vi "Test Read-Write Control Text.vi"(8 "error in (no error)":errorcluster) -> (0 "error out":errorcluster, 3 "Pass?":bool)   [LabVIEW 2020]
uses:
  G-Unicode/Unicode/Controls/String Encoding.ctl
  G-Unicode/Types/UTF-8 String/UTF-8 String.lvclass/UTF-8 String.ctl
  5655a432-7152-4618-8a1b-1a6feeb00f3f.vi
  G-Unicode/Dialog & User Interface/Polymorphic VIs/Write Control Text/Write Listbox Header (UTF-8 String).vi
  G-Unicode/Dialog & User Interface/Polymorphic VIs/Read Control Text/Read Listbox Header (UTF-8 String).vi
  47e1521e-4900-4e50-93d0-971907de44b7.vi
  G-Unicode/Dialog & User Interface/Polymorphic VIs/Write Control Text/Write Graph Plot Names (UTF-8 String).vi
  G-Unicode/Dialog & User Interface/Polymorphic VIs/Write Control Text/Write Graph Cursor Names (UTF-8 String).vi
  G-Unicode/Dialog & User Interface/Polymorphic VIs/Write Control Text/Write Graph Axis Labels (UTF-8 String).vi
  G-Unicode/Dialog & User Interface/Polymorphic VIs/Write Control Text/Write Table Headers (UTF-8 String).vi
  G-Unicode/Dialog & User Interface/Polymorphic VIs/Read Control Text/Read Table Headers (UTF-8 String).vi
  cbd299b7-ed5c-44d8-98e3-4b07b256a3af.vi
  97e6e9dd-fb41-465e-8130-768105b8566a.vi
  G-Unicode/Dialog & User Interface/Polymorphic VIs/Write Control Text/Write Multicolumn Listbox Headers (UTF-8 String).vi
  G-Unicode/Dialog & User Interface/Polymorphic VIs/Read Control Text/Read Multicolumn Listbox Headers (UTF-8 String).vi
  2cb1db3a-9545-49da-8e46-b28431192bfb.vi
  d3ca7cbe-fe55-4c08-9226-8df1279bea32.vi
  G-Unicode/Dialog & User Interface/Polymorphic VIs/Write Control Text/Write Radio Button Text (UTF-8 String).vi
  G-Unicode/Dialog & User Interface/Polymorphic VIs/Read Control Text/Read Radio Button Text (UTF-8 String).vi
  c66c8a8e-6384-46dd-ad34-c6b36e981c5f.vi
  G-Unicode/Dialog & User Interface/Polymorphic VIs/Write Control Text/Write Tab Pages (UTF-8 String).vi
  G-Unicode/Dialog & User Interface/Polymorphic VIs/Read Control Text/Read Tab Pages (UTF-8 String).vi
  11ce0e2c-e1a8-46a3-af78-7df26efc8245.vi
  G-Unicode/Dialog & User Interface/Polymorphic VIs/Write Control Text/Write Listbox Items (UTF-8 String).vi
  G-Unicode/Dialog & User Interface/Polymorphic VIs/Read Control Text/Read Listbox Items (UTF-8 String).vi
  c5b5f753-7993-4590-ab7a-38cd070e680f.vi
  G-Unicode/Dialog & User Interface/Polymorphic VIs/Write Control Text/Write Table Value (UTF-8 String).vi
  G-Unicode/Dialog & User Interface/Polymorphic VIs/Read Control Text/Read Table Value (UTF-8 String).vi
  d87d6912-68ee-4c4f-8e1f-9eaf2c3e8737.vi
  G-Unicode/Dialog & User Interface/Polymorphic VIs/Write Control Text/Write Ring Strings (UTF-8 String).vi
  G-Unicode/Dialog & User Interface/Polymorphic VIs/Read Control Text/Read Ring Strings (UTF-8 String).vi
  b51df372-b908-46a9-9cd9-1bce9bcba761.vi
  3f50c59c-438d-4159-8265-e7e5e4819d1d.vi
  G-Unicode/Dialog & User Interface/Polymorphic VIs/Write Control Text/Write 2D String Array Value (UTF-8 String).vi
  G-Unicode/Dialog & User Interface/Polymorphic VIs/Read Control Text/Read 2D String Array Value (UTF-8 String).vi
  f481c7ac-37a4-4879-9d59-93dd94c77838.vi
  G-Unicode/Dialog & User Interface/Polymorphic VIs/Write Control Text/Write 1D String Array Value (UTF-8 String).vi
  G-Unicode/Dialog & User Interface/Polymorphic VIs/Read Control Text/Read 1D String Array Value (UTF-8 String).vi
  2abff34c-ba54-40bb-bfb0-e7a9eb1a66c8.vi
  G-Unicode/Dialog & User Interface/Polymorphic VIs/Write Control Text/Write String Value (UTF-8 String).vi
  G-Unicode/Dialog & User Interface/Polymorphic VIs/Read Control Text/Read String Value (UTF-8 String).vi
  b9bba32d-5ca2-4258-b841-0da24b58b874.vi
  G-Unicode/Dialog & User Interface/Polymorphic VIs/Write Control Text/Write Multicolumn Listbox Items (UTF-8 String).vi
  G-Unicode/Dialog & User Interface/Polymorphic VIs/Read Control Text/Read Multicolumn Listbox Items (UTF-8 String).vi
  4c20338b-6e60-4a75-91ad-9e96f58f92b0.vi
  G-Unicode/Unicode/Encode String.vi
  5655a432-7152-4618-8a1b-1a6feeb00f3f.vi/46bf550a-28c6-4dfd-813a-9b0ad34779ef.vi
  G-Unicode/Private/Conversion/String as Encoded String.vi
  G-Unicode/Private/Conversion/Polymorphic VIs/String as Encoded String (UTF-8 String).vi
  G-Unicode/Types/UTF-8 String/Write Encoded UTF-8 String.vi
  G-Unicode/Dialog & User Interface/Polymorphic VIs/Write Control Text/Write Listbox Header (UTF-8 String).vi/5206cb6b-04fb-41f5-a37e-29c14f142303.vi
  G-Unicode/Dialog & User Interface/Polymorphic VIs/Read Control Text/Read Listbox Header (UTF-8 String).vi/bfba3187-b22e-4285-8cc2-1816a803f974.vi
  47e1521e-4900-4e50-93d0-971907de44b7.vi/3a31b270-3bb6-4c58-a256-c5fcc2c98f09.vi
  47e1521e-4900-4e50-93d0-971907de44b7.vi/0ec5df2d-ef9b-4f84-a6a8-ffcedd45c4dc.vi
  G-Unicode/Dialog & User Interface/Polymorphic VIs/Write Control Text/Write Graph Plot Names (UTF-8 String).vi/5206cb6b-04fb-41f5-a37e-29c14f142303.vi
  G-Unicode/Dialog & User Interface/Polymorphic VIs/Write Control Text/Write Graph Cursor Names (UTF-8 String).vi/5206cb6b-04fb-41f5-a37e-29c14f142303.vi
  G-Unicode/Dialog & User Interface/Polymorphic VIs/Write Control Text/Write Graph Axis Labels (UTF-8 String).vi/5206cb6b-04fb-41f5-a37e-29c14f142303.vi
  G-Unicode/Dialog & User Interface/Polymorphic VIs/Write Control Text/Write Graph Axis Labels (UTF-8 String).vi/dd8e371b-806c-4d03-8f90-d02a4c0388fb.vi
  G-Unicode/Dialog & User Interface/Polymorphic VIs/Write Control Text/Write Table Headers (UTF-8 String).vi/5206cb6b-04fb-41f5-a37e-29c14f142303.vi
  G-Unicode/Dialog & User Interface/Polymorphic VIs/Write Control Text/Write Table Headers (UTF-8 String).vi/ac01c1c3-6448-4046-bb74-48d1977bc508.vi
  G-Unicode/Dialog & User Interface/Polymorphic VIs/Read Control Text/Read Table Headers (UTF-8 String).vi/f6f7f231-7ddf-476b-a943-0386d848a5c9.vi
  G-Unicode/Dialog & User Interface/Polymorphic VIs/Read Control Text/Read Table Headers (UTF-8 String).vi/fba5a6d2-cdfe-4afc-9e2c-d2641906be0d.vi
  cbd299b7-ed5c-44d8-98e3-4b07b256a3af.vi/3a31b270-3bb6-4c58-a256-c5fcc2c98f09.vi
  cbd299b7-ed5c-44d8-98e3-4b07b256a3af.vi/0ec5df2d-ef9b-4f84-a6a8-ffcedd45c4dc.vi
  97e6e9dd-fb41-465e-8130-768105b8566a.vi/3a31b270-3bb6-4c58-a256-c5fcc2c98f09.vi
  97e6e9dd-fb41-465e-8130-768105b8566a.vi/0ec5df2d-ef9b-4f84-a6a8-ffcedd45c4dc.vi
  G-Unicode/Dialog & User Interface/Polymorphic VIs/Write Control Text/Write Multicolumn Listbox Headers (UTF-8 String).vi/5206cb6b-04fb-41f5-a37e-29c14f142303.vi
  G-Unicode/Dialog & User Interface/Polymorphic VIs/Write Control Text/Write Multicolumn Listbox Headers (UTF-8 String).vi/ac01c1c3-6448-4046-bb74-48d1977bc508.vi
  G-Unicode/Dialog & User Interface/Polymorphic VIs/Read Control Text/Read Multicolumn Listbox Headers (UTF-8 String).vi/f6f7f231-7ddf-476b-a943-0386d848a5c9.vi
  G-Unicode/Dialog & User Interface/Polymorphic VIs/Read Control Text/Read Multicolumn Listbox Headers (UTF-8 String).vi/fba5a6d2-cdfe-4afc-9e2c-d2641906be0d.vi
  2cb1db3a-9545-49da-8e46-b28431192bfb.vi/3a31b270-3bb6-4c58-a256-c5fcc2c98f09.vi
  2cb1db3a-9545-49da-8e46-b28431192bfb.vi/0ec5df2d-ef9b-4f84-a6a8-ffcedd45c4dc.vi
  d3ca7cbe-fe55-4c08-9226-8df1279bea32.vi/3a31b270-3bb6-4c58-a256-c5fcc2c98f09.vi
  d3ca7cbe-fe55-4c08-9226-8df1279bea32.vi/0ec5df2d-ef9b-4f84-a6a8-ffcedd45c4dc.vi
  G-Unicode/Dialog & User Interface/Polymorphic VIs/Write Control Text/Write Radio Button Text (UTF-8 String).vi/5206cb6b-04fb-41f5-a37e-29c14f142303.vi
  G-Unicode/Dialog & User Interface/Polymorphic VIs/Read Control Text/Read Radio Button Text (UTF-8 String).vi/f6f7f231-7ddf-476b-a943-0386d848a5c9.vi
  c66c8a8e-6384-46dd-ad34-c6b36e981c5f.vi/3a31b270-3bb6-4c58-a256-c5fcc2c98f09.vi
  c66c8a8e-6384-46dd-ad34-c6b36e981c5f.vi/0ec5df2d-ef9b-4f84-a6a8-ffcedd45c4dc.vi
  G-Unicode/Dialog & User Interface/Polymorphic VIs/Write Control Text/Write Tab Pages (UTF-8 String).vi/5206cb6b-04fb-41f5-a37e-29c14f142303.vi
  G-Unicode/Dialog & User Interface/Polymorphic VIs/Read Control Text/Read Tab Pages (UTF-8 String).vi/f6f7f231-7ddf-476b-a943-0386d848a5c9.vi
  11ce0e2c-e1a8-46a3-af78-7df26efc8245.vi/3a31b270-3bb6-4c58-a256-c5fcc2c98f09.vi
  11ce0e2c-e1a8-46a3-af78-7df26efc8245.vi/0ec5df2d-ef9b-4f84-a6a8-ffcedd45c4dc.vi
  G-Unicode/Dialog & User Interface/Polymorphic VIs/Write Control Text/Write Listbox Items (UTF-8 String).vi/5206cb6b-04fb-41f5-a37e-29c14f142303.vi
  G-Unicode/Dialog & User Interface/Polymorphic VIs/Read Control Text/Read Listbox Items (UTF-8 String).vi/f6f7f231-7ddf-476b-a943-0386d848a5c9.vi
  c5b5f753-7993-4590-ab7a-38cd070e680f.vi/3a31b270-3bb6-4c58-a256-c5fcc2c98f09.vi
  c5b5f753-7993-4590-ab7a-38cd070e680f.vi/0ec5df2d-ef9b-4f84-a6a8-ffcedd45c4dc.vi
  G-Unicode/Dialog & User Interface/Polymorphic VIs/Write Control Text/Write Table Value (UTF-8 String).vi/5206cb6b-04fb-41f5-a37e-29c14f142303.vi
  G-Unicode/Dialog & User Interface/Polymorphic VIs/Read Control Text/Read Table Value (UTF-8 String).vi/f6f7f231-7ddf-476b-a943-0386d848a5c9.vi
  d87d6912-68ee-4c4f-8e1f-9eaf2c3e8737.vi/3a31b270-3bb6-4c58-a256-c5fcc2c98f09.vi
  d87d6912-68ee-4c4f-8e1f-9eaf2c3e8737.vi/0ec5df2d-ef9b-4f84-a6a8-ffcedd45c4dc.vi
  G-Unicode/Dialog & User Interface/Polymorphic VIs/Write Control Text/Write Ring Strings (UTF-8 String).vi/5206cb6b-04fb-41f5-a37e-29c14f142303.vi
  G-Unicode/Dialog & User Interface/Polymorphic VIs/Read Control Text/Read Ring Strings (UTF-8 String).vi/f6f7f231-7ddf-476b-a943-0386d848a5c9.vi
  b51df372-b908-46a9-9cd9-1bce9bcba761.vi/3a31b270-3bb6-4c58-a256-c5fcc2c98f09.vi
  b51df372-b908-46a9-9cd9-1bce9bcba761.vi/0ec5df2d-ef9b-4f84-a6a8-ffcedd45c4dc.vi
  3f50c59c-438d-4159-8265-e7e5e4819d1d.vi/3a31b270-3bb6-4c58-a256-c5fcc2c98f09.vi
  3f50c59c-438d-4159-8265-e7e5e4819d1d.vi/0ec5df2d-ef9b-4f84-a6a8-ffcedd45c4dc.vi
  G-Unicode/Dialog & User Interface/Polymorphic VIs/Write Control Text/Write 2D String Array Value (UTF-8 String).vi/5206cb6b-04fb-41f5-a37e-29c14f142303.vi
  G-Unicode/Dialog & User Interface/Polymorphic VIs/Read Control Text/Read 2D String Array Value (UTF-8 String).vi/f6f7f231-7ddf-476b-a943-0386d848a5c9.vi
  f481c7ac-37a4-4879-9d59-93dd94c77838.vi/3a31b270-3bb6-4c58-a256-c5fcc2c98f09.vi
  f481c7ac-37a4-4879-9d59-93dd94c77838.vi/0ec5df2d-ef9b-4f84-a6a8-ffcedd45c4dc.vi
  G-Unicode/Dialog & User Interface/Polymorphic VIs/Write Control Text/Write 1D String Array Value (UTF-8 String).vi/5206cb6b-04fb-41f5-a37e-29c14f142303.vi
  G-Unicode/Dialog & User Interface/Polymorphic VIs/Read Control Text/Read 1D String Array Value (UTF-8 String).vi/f6f7f231-7ddf-476b-a943-0386d848a5c9.vi
  2abff34c-ba54-40bb-bfb0-e7a9eb1a66c8.vi/3a31b270-3bb6-4c58-a256-c5fcc2c98f09.vi
  2abff34c-ba54-40bb-bfb0-e7a9eb1a66c8.vi/0ec5df2d-ef9b-4f84-a6a8-ffcedd45c4dc.vi
  G-Unicode/Dialog & User Interface/Polymorphic VIs/Write Control Text/Write String Value (UTF-8 String).vi/5206cb6b-04fb-41f5-a37e-29c14f142303.vi
  G-Unicode/Dialog & User Interface/Polymorphic VIs/Read Control Text/Read String Value (UTF-8 String).vi/bfba3187-b22e-4285-8cc2-1816a803f974.vi
  b9bba32d-5ca2-4258-b841-0da24b58b874.vi/3a31b270-3bb6-4c58-a256-c5fcc2c98f09.vi
  b9bba32d-5ca2-4258-b841-0da24b58b874.vi/0ec5df2d-ef9b-4f84-a6a8-ffcedd45c4dc.vi
  G-Unicode/Dialog & User Interface/Polymorphic VIs/Write Control Text/Write Multicolumn Listbox Items (UTF-8 String).vi/5206cb6b-04fb-41f5-a37e-29c14f142303.vi
  G-Unicode/Dialog & User Interface/Polymorphic VIs/Read Control Text/Read Multicolumn Listbox Items (UTF-8 String).vi/f6f7f231-7ddf-476b-a943-0386d848a5c9.vi
  4c20338b-6e60-4a75-91ad-9e96f58f92b0.vi/3a31b270-3bb6-4c58-a256-c5fcc2c98f09.vi
  4c20338b-6e60-4a75-91ad-9e96f58f92b0.vi/0ec5df2d-ef9b-4f84-a6a8-ffcedd45c4dc.vi
  G-Unicode/Private/Conversion/Text to UTF-8.vi
  G-Unicode/Private/Conversion/Polymorphic VIs/Text to UTF-8 (LabVIEW String).vi
  G-Unicode/Private/Conversion/Encoded UTF-8 String to Encoded UTF-16LE String.vi
  G-Unicode/Unicode/SubVIs/UTF-16 Byte Swap.vi
  G-Unicode/Private/Conversion/UTF-8 to Text.vi
  G-Unicode/Private/Conversion/Polymorphic VIs/UTF-8 to Text (LabVIEW String).vi
  G-Unicode/Private/Conversion/Encoded UTF-16LE String to Encoded UTF-8 String.vi
  G-Unicode/Unicode/Prepend BOM.vi
  G-Unicode/Private/Conversion/Polymorphic VIs/String as Encoded String (LabVIEW String).vi
  G-Unicode/Types/UTF-8 String/Read Encoded UTF-8 String.vi
  G-Unicode/Private/Conversion/Text as Encoded String.vi
  G-Unicode/Private/Conversion/Polymorphic VIs/Text as Encoded String (UTF-8 String).vi
  G-Unicode/Unicode/SubVIs/Byte Order Marks.vi
  G-Unicode/Unicode/Detect BOM.vi
  G-Unicode/Unicode/Detect String Encoding.vi
  G-Unicode/Private/User Interface/Write String.vi
  G-Unicode/Private/User Interface/Read String.vi
  G-Unicode/Private/User Interface/Write String Array (1D).vi
  G-Unicode/Private/User Interface/Read String Array (1D).vi
  G-Unicode/Private/User Interface/Write String Array (2D).vi
  G-Unicode/Private/User Interface/Read String Array (2D).vi
  G-Unicode/Private/User Interface/Write Ring Control.vi
  G-Unicode/Private/User Interface/Read Ring Control.vi
  G-Unicode/Private/User Interface/Write MultCol Listbox Data.vi
  G-Unicode/Private/User Interface/Read MultCol Listbox Data.vi
  G-Unicode/Private/User Interface/Write MultCol Listbox Headers.vi
  G-Unicode/Private/User Interface/Read MultCol Listbox Headers.vi
  G-Unicode/Private/User Interface/Write Listbox Data.vi
  G-Unicode/Private/User Interface/Read Listbox Data.vi
  G-Unicode/Private/User Interface/Write Listbox Header.vi
  G-Unicode/Private/User Interface/Read Listbox Header.vi
  G-Unicode/Private/User Interface/Write Table Data.vi
  G-Unicode/Private/User Interface/Read Table Data.vi
  G-Unicode/Private/User Interface/Write Table Headers.vi
  G-Unicode/Private/User Interface/Read Table Headers.vi
  G-Unicode/Private/User Interface/Write Tab Control.vi
  G-Unicode/Private/User Interface/Read Tab Control.vi
  G-Unicode/Private/User Interface/Write Radio Buttons.vi
  G-Unicode/Private/User Interface/Read Radio Button Text.vi
  G-Unicode/Private/User Interface/Write Graph-Chart Plot Names.vi
  G-Unicode/Private/User Interface/Write Graph-Chart Axis Labels.vi
  G-Unicode/Private/User Interface/Write Graph-Chart Cursor Names.vi
  G-Unicode/Types/UTF-8 String/UTF-8 String.lvclass
  G-Unicode/G-Unicode.lvlib
panel:
  out "Waveform Graph":dbl[](graph)
  out "Waveform Chart":dbl(graph)
  in  "Radio Buttons":T1(radio)
  in  "Tab Control":enum32{"Page 1", "Page 2", "Page 3", "Page 4"}(tab)
  in  "Multicolumn Listbox":i32(listbox)
  in  "Listbox":i32(listbox)
  in  "Table Control":string[][](table)
  in  "Menu Ring":u16(ring)
  in  "Text Ring":u16(ring)
  in  "String Array (2D)":string[][](array[string])
  in  "String Array (1D)":string[](array[string])
  in  "String":string
  # "Note the dropdowns for the ring controls aren't rendered correctly, but when selected it looks OK."
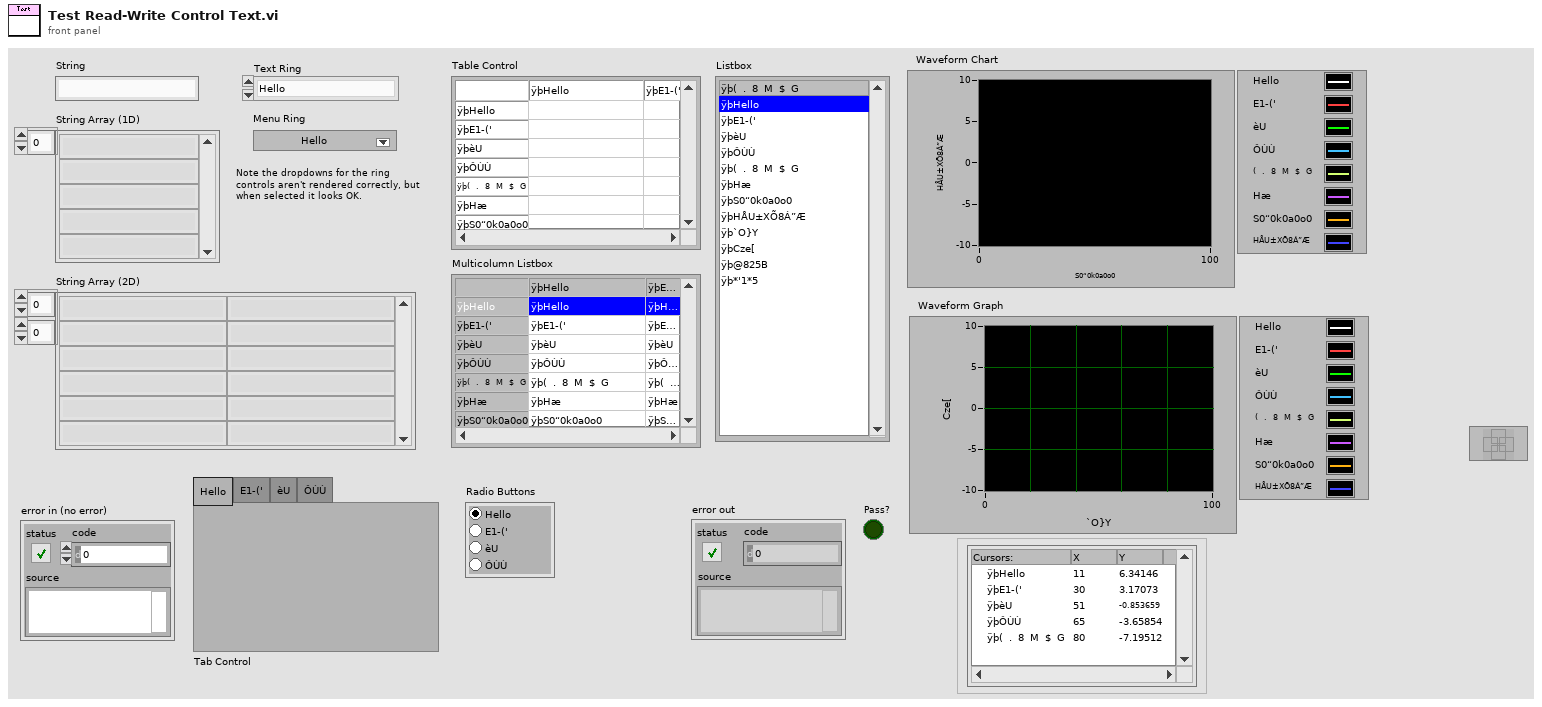
[diagram p1: front panel]
types:
  T1 = enum32{"Radio Selection 1", "Radio Selection 2", "Radio Selection 3", "Radio Selection 4"}
  T2 = typedef "G-Unicode.lvlib/String Encoding.ctl" = enum16{"ANSI", "UTF-8", "UTF-16LE", "UTF-16BE", "Unknown"}
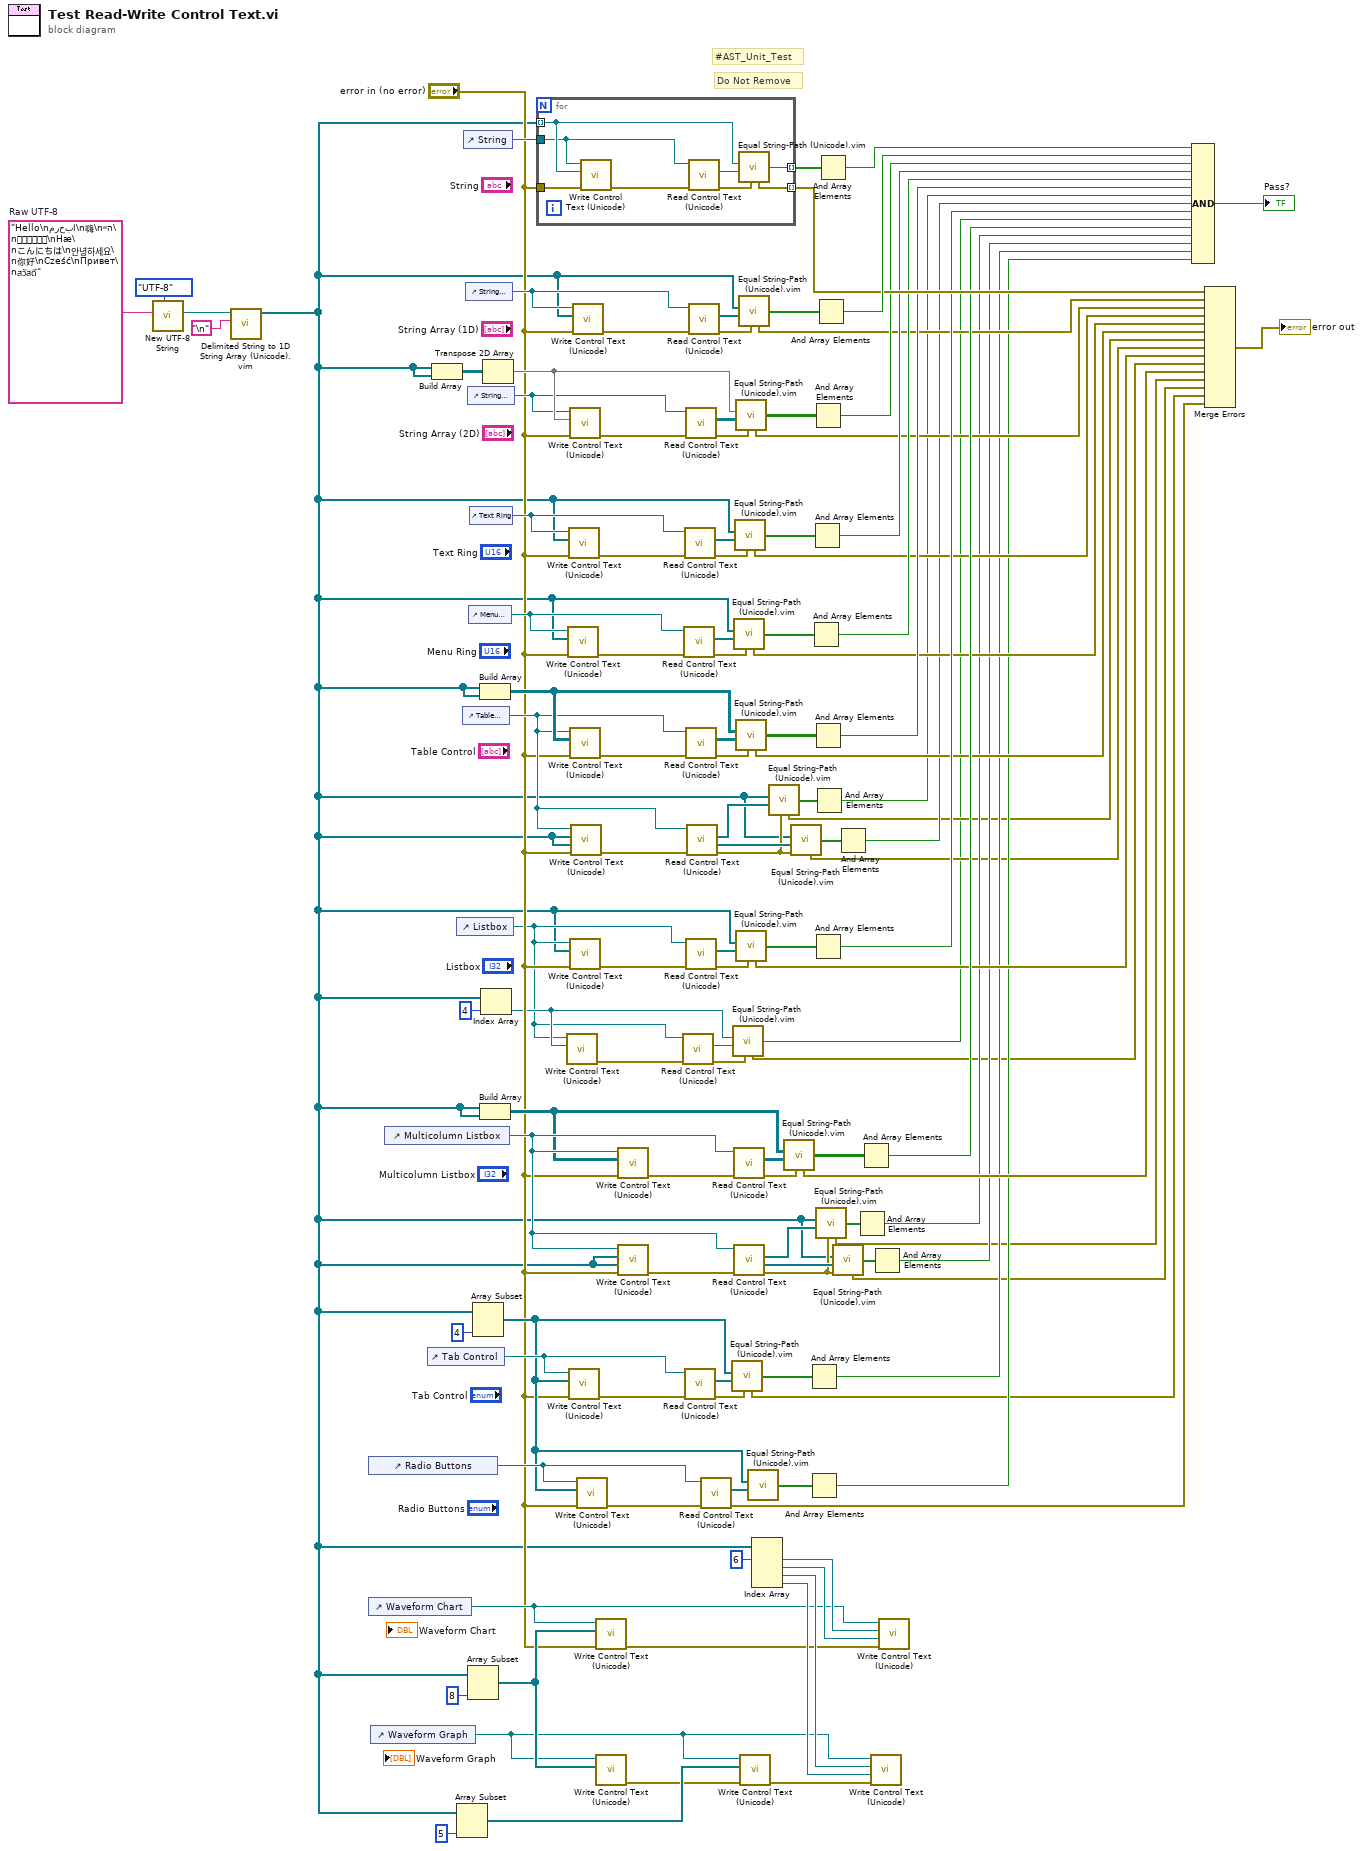
[diagram p0: block diagram]
diagram:
  w2 = "Hello\nمرحبا\n嗨\nהיי\nनमस्ते\nHæ\nこんにちは\n안녕하세요\n你好\nCześć\nПривет\nสวัสดี"  # Raw UTF-8
  # "Do Not Remove"
  # "#AST_Unit_Test"
  n1 = call "New UTF-8 String.vi"("Input Encoding (ANSI)"=String_Encoding."UTF-8", "String"=w2) -> ("UTF-8 String"=w4:refnum<class "UTF-8 String.lvclass">)  [unwired: 8 in, 1 out]
  n2 = call "Delimited String to 1D String Array (Unicode).vim"("Delimiter (tab)"="\n", "Delimited String"=w4) -> ("String Array"=w1:refnum<class "UTF-8 String.lvclass">[])  [unwired: 8 in, 1 out]
  n3 = control-ref of="Radio Buttons"() -> (w44:refnum<vi>)
  n4 = control-ref of="Waveform Chart"() -> (w52:refnum<vi>)
  n5 = control-ref of="Waveform Graph"() -> (w56:refnum<vi>)
  n6 = control-ref of="Multicolumn Listbox"() -> (w41:refnum<vi>)
  n7 = control-ref of="Tab Control"() -> (w47:refnum<vi>)
  n8 = Build Array(w1, w1) -> (w108:refnum<class "UTF-8 String.lvclass">[][])
  n9 = control-ref of="Listbox"() -> (w8:refnum<vi>)
  n10 = Array Subset(array=w1, length=5) -> (w64:refnum<class "UTF-8 String.lvclass">[])  [unwired: 1 in]
  n11 = control-ref of="Table Control"() -> (w26:refnum<vi>)
  n12 = control-ref of="String"() -> (w121:refnum<vi>)
  n13 = control-ref of="String Array (1D)"() -> (w51:refnum<vi>)
  n14 = control-ref of="String Array (2D)"() -> (w50:refnum<vi>)
  n15 = Array Subset(array=w1, length=8) -> (w62:refnum<class "UTF-8 String.lvclass">[])  [unwired: 1 in]
  n16 = control-ref of="Menu Ring"() -> (w48:refnum<vi>)
  n17 = control-ref of="Text Ring"() -> (w49:refnum<vi>)
  n18 = Array Subset(array=w1, length=4) -> (w43:refnum<class "UTF-8 String.lvclass">[])  [unwired: 1 in]
  n19 = Build Array(w1, w1) -> (w94:refnum<class "UTF-8 String.lvclass">[][])
  n20 = Build Array(w1, w1) -> (w40:refnum<class "UTF-8 String.lvclass">[][])
  n21 = Index Array(array=w1, index=4) -> (element=w9:refnum<class "UTF-8 String.lvclass">)
  n22 = Transpose 2D Array(2D array=w108) -> (transposed array=w106:refnum<class "UTF-8 String.lvclass">[][])
  n23 = for {
    tunnel: w121 -> [w122]
    tunnel: w1 -> [w124] mode=indexing
    tunnel: "error in (no error)" -> [w128]
    tunnel: [w125] -> w112 mode=indexing
    tunnel: [w127] -> w120 mode=indexing
    n24 = call-poly "Write Control Text (Unicode).vi"("error in"=w128, "Value"=w124, "Control Ref"=w122) -> ("error out"=w123:errorcluster)  [unwired: 8 in]
    n25 = call-poly "Read Control Text (Unicode).vi"("error in"=w123, "Control Ref"=w122) -> ("error out"=w126:errorcluster, "UTF-8 String"=w129:refnum<class "UTF-8 String.lvclass">)  [unwired: 8 in]
    n26 = call "Equal String-Path (Unicode).vim"("error in"=w126, "y"=w129, "x"=w124) -> ("error out"=w125:errorcluster, "Equal?"=w127:bool)  [unwired: 6 in]
  }
  n27 = call-poly "Write Control Text (Unicode).vi"("Value"=w9, "Control Ref"=w8) -> ("error out"=w13:errorcluster)  [unwired: 9 in]
  n28 = call-poly "Write Control Text (Unicode).vi"("error in"="error in (no error)", "Value"=w1, "Control Ref"=w48) -> ("error out"=w102:errorcluster)  [unwired: 8 in]
  n29 = call-poly "Write Control Text (Unicode).vi"("error in"="error in (no error)", "Value"=w1, "Control Ref"=w49) -> ("error out"=w103:errorcluster)  [unwired: 8 in]
  n30 = call-poly "Write Control Text (Unicode).vi"("error in"="error in (no error)", "Value"=w43, "Control Ref"=w47) -> ("error out"=w69:errorcluster)  [unwired: 8 in]
  n31 = call-poly "Write Control Text (Unicode).vi"("error in"="error in (no error)", "Value"=w106, "Control Ref"=w50) -> ("error out"=w110:errorcluster)  [unwired: 8 in]
  n32 = call-poly "Write Control Text (Unicode).vi"("error in"="error in (no error)", "Value"=w94, "Control Ref"=w26) -> ("error out"=w96:errorcluster)  [unwired: 8 in]
  n33 = call-poly "Write Control Text (Unicode).vi"("error in"="error in (no error)", "Value"=w1, "Control Ref"=w8) -> ("error out"=w90:errorcluster)  [unwired: 8 in]
  n34 = call-poly "Write Control Text (Unicode).vi"("error in"="error in (no error)", "Row Headers"=w1, "Column Headers"=w1, "Control Ref"=w26) -> ("error out"=w28:errorcluster)  [unwired: 7 in]
  n35 = call-poly "Write Control Text (Unicode).vi"("error in"="error in (no error)", "Value"=w1, "Control Ref"=w51) -> ("error out"=w115:errorcluster)  [unwired: 8 in]
  n36 = call-poly "Write Control Text (Unicode).vi"("error in"="error in (no error)", "Value"=w43, "Control Ref"=w44) -> ("error out"=w45:errorcluster)  [unwired: 8 in]
  n37 = call-poly "Write Control Text (Unicode).vi"("error in"="error in (no error)", "Plot Names"=w62, "Control Ref"=w52) -> ("error out"=w53:errorcluster)  [unwired: 8 in]
  n38 = call-poly "Write Control Text (Unicode).vi"("Plot Names"=w62, "Control Ref"=w56) -> ("error out"=w55:errorcluster)  [unwired: 9 in]
  n39 = call-poly "Write Control Text (Unicode).vi"("error in"="error in (no error)", "Value"=w40, "Control Ref"=w41) -> ("error out"=w87:errorcluster)  [unwired: 8 in]
  n40 = call-poly "Write Control Text (Unicode).vi"("error in"="error in (no error)", "Row Headers"=w1, "Column Headers"=w1, "Control Ref"=w41) -> ("error out"=w37:errorcluster)  [unwired: 7 in]
  n41 = call-poly "Read Control Text (Unicode).vi"("error in"=w13, "Control Ref"=w8) -> ("error out"=w12:errorcluster, "Value"=w11:refnum<class "UTF-8 String.lvclass">)  [unwired: 8 in]
  n42 = call-poly "Read Control Text (Unicode).vi"("error in"=w102, "Control Ref"=w48) -> ("error out"=w76:errorcluster, "Value"=w101:refnum<class "UTF-8 String.lvclass">[])  [unwired: 8 in]
  n43 = call-poly "Read Control Text (Unicode).vi"("error in"=w103, "Control Ref"=w49) -> ("error out"=w78:errorcluster, "Value"=w104:refnum<class "UTF-8 String.lvclass">[])  [unwired: 8 in]
  n44 = call-poly "Read Control Text (Unicode).vi"("error in"=w69, "Control Ref"=w47) -> ("error out"=w67:errorcluster, "Value"=w68:refnum<class "UTF-8 String.lvclass">[])  [unwired: 8 in]
  n45 = call-poly "Read Control Text (Unicode).vi"("error in"=w110, "Control Ref"=w50) -> ("error out"=w80:errorcluster, "Value"=w109:refnum<class "UTF-8 String.lvclass">[][])  [unwired: 8 in]
  n46 = call-poly "Read Control Text (Unicode).vi"("error in"=w96, "Control Ref"=w26) -> ("error out"=w74:errorcluster, "Value"=w97:refnum<class "UTF-8 String.lvclass">[][])  [unwired: 8 in]
  n47 = call-poly "Read Control Text (Unicode).vi"("error in"=w90, "Control Ref"=w8) -> ("error out"=w72:errorcluster, "Value"=w91:refnum<class "UTF-8 String.lvclass">[])  [unwired: 8 in]
  n48 = call-poly "Read Control Text (Unicode).vi"("error in"=w28, "Control Ref"=w26) -> ("error out"=w16:errorcluster, "Row Headers"=w25:refnum<class "UTF-8 String.lvclass">[], "Column Headers"=w27:refnum<class "UTF-8 String.lvclass">[])  [unwired: 7 in]
  n49 = call-poly "Read Control Text (Unicode).vi"("error in"=w115, "Control Ref"=w51) -> ("error out"=w82:errorcluster, "Value"=w116:refnum<class "UTF-8 String.lvclass">[])  [unwired: 8 in]
  n50 = call-poly "Read Control Text (Unicode).vi"("error in"=w45, "Control Ref"=w44) -> ("error out"=w29:errorcluster, "Value"=w46:refnum<class "UTF-8 String.lvclass">[])  [unwired: 8 in]
  n51 = call "Equal String-Path (Unicode).vim"("error in"=w67, "y"=w68, "x"=w43) -> ("error out"=w30:errorcluster, "Equal?"=w66:bool[])  [unwired: 6 in]
  n52 = call "Equal String-Path (Unicode).vim"("error in"=w12, "y"=w11, "x"=w9) -> ("error out"=w6:errorcluster, "Equal?"=w7:bool)  [unwired: 6 in]
  n53 = call "Equal String-Path (Unicode).vim"("error in"=w76, "y"=w101, "x"=w1) -> ("error out"=w75:errorcluster, "Equal?"=w100:bool[])  [unwired: 6 in]
  n54 = call-poly "Read Control Text (Unicode).vi"("error in"=w87, "Control Ref"=w41) -> ("error out"=w84:errorcluster, "Value"=w86:refnum<class "UTF-8 String.lvclass">[][])  [unwired: 8 in]
  n55 = call-poly "Read Control Text (Unicode).vi"("error in"=w37, "Control Ref"=w41) -> ("error out"=w19:errorcluster, "Row Headers"=w38:refnum<class "UTF-8 String.lvclass">[], "Column Headers"=w39:refnum<class "UTF-8 String.lvclass">[])  [unwired: 7 in]
  n56 = call "Equal String-Path (Unicode).vim"("error in"=w78, "y"=w104, "x"=w1) -> ("error out"=w77:errorcluster, "Equal?"=w105:bool[])  [unwired: 6 in]
  n57 = call "Equal String-Path (Unicode).vim"("error in"=w80, "y"=w109, "x"=w106) -> ("error out"=w79:errorcluster, "Equal?"=w111:bool[][])  [unwired: 6 in]
  n58 = call "Equal String-Path (Unicode).vim"("error in"=w74, "y"=w97, "x"=w94) -> ("error out"=w73:errorcluster, "Equal?"=w95:bool[][])  [unwired: 6 in]
  n59 = call "Equal String-Path (Unicode).vim"("error in"=w72, "y"=w91, "x"=w1) -> ("error out"=w71:errorcluster, "Equal?"=w92:bool[])  [unwired: 6 in]
  n60 = call "Equal String-Path (Unicode).vim"("error in"=w82, "y"=w116, "x"=w1) -> ("error out"=w81:errorcluster, "Equal?"=w114:bool[])  [unwired: 6 in]
  n61 = call-poly "Write Control Text (Unicode).vi"("error in"=w55, "Cursor Names"=w64, "Control Ref"=w56) -> ("error out"=w54:errorcluster)  [unwired: 8 in]
  n62 = call "Equal String-Path (Unicode).vim"("y"=w46, "x"=w43) -> ("Equal?"=w42:bool[])  [unwired: 7 in, 1 out]
  n63 = Index Array(array=w1, index #1=6 ("index")) -> (element #1=w60:refnum<class "UTF-8 String.lvclass">, element #2=w59:refnum<class "UTF-8 String.lvclass">, element #3=w58:refnum<class "UTF-8 String.lvclass">, element #4=w57:refnum<class "UTF-8 String.lvclass">)  [unwired: 3 in]
  n64 = call "Equal String-Path (Unicode).vim"("error in"=w16, "y"=w27, "x"=w1) -> ("error out"=w14:errorcluster, "Equal?"=w24:bool[])  [unwired: 6 in]
  n65 = call "Equal String-Path (Unicode).vim"("error in"=w84, "y"=w86, "x"=w40) -> ("error out"=w83:errorcluster, "Equal?"=w88:bool[][])  [unwired: 6 in]
  n66 = call "Equal String-Path (Unicode).vim"("error in"=w16, "y"=w25, "x"=w1) -> ("error out"=w15:errorcluster, "Equal?"=w23:bool[])  [unwired: 6 in]
  n67 = And Array Elements(Boolean array=w66) -> (logical AND=w33:bool)
  n68 = And Array Elements(Boolean array=w42) -> (logical AND=w34:bool)
  n69 = And Array Elements(Boolean array=w100) -> (logical AND=w98:bool)
  n70 = And Array Elements(Boolean array=w105) -> (logical AND=w99:bool)
  n71 = And Array Elements(Boolean array=w111) -> (logical AND=w107:bool)
  n72 = And Array Elements(Boolean array=w95) -> (logical AND=w93:bool)
  n73 = And Array Elements(Boolean array=w92) -> (logical AND=w89:bool)
  n74 = And Array Elements(Boolean array=w24) -> (logical AND=w22:bool)
  n75 = And Array Elements(Boolean array=w114) -> (logical AND=w113:bool)
  n76 = call "Equal String-Path (Unicode).vim"("error in"=w19, "y"=w39, "x"=w1) -> ("error out"=w17:errorcluster, "Equal?"=w36:bool[])  [unwired: 6 in]
  n77 = And Array Elements(Boolean array=w120) -> (logical AND=w119:bool)
  n78 = call "Equal String-Path (Unicode).vim"("error in"=w19, "y"=w38, "x"=w1) -> ("error out"=w18:errorcluster, "Equal?"=w35:bool[])  [unwired: 6 in]
  n79 = And Array Elements(Boolean array=w23) -> (logical AND=w21:bool)
  n80 = And Array Elements(Boolean array=w36) -> (logical AND=w32:bool)
  n81 = And Array Elements(Boolean array=w88) -> (logical AND=w85:bool)
  n82 = call-poly "Write Control Text (Unicode).vi"("error in"=w54, "Y Axis"=w57, "X Axis"=w58, "Control Ref"=w56) -> ()  [unwired: 7 in, 1 out]
  n83 = And Array Elements(Boolean array=w35) -> (logical AND=w31:bool)
  n84 = call-poly "Write Control Text (Unicode).vi"("error in"=w53, "Y Axis"=w59, "X Axis"=w60, "Control Ref"=w52) -> ()  [unwired: 7 in, 1 out]
  n85 = Compound Arithmetic op=AND(w119, w113, w107, w99, w98, w93, w22, w21, w89, w7, w85, w32, w31, w33, w34) -> (→"Pass?":bool)
  n86 = Merge Errors(w112, w81, w79, w77, w75, w73, w14, w15, w71, w6, w83, w17, w18, w30, w29) -> (→"error out":errorcluster)
